vi "NISearchDLGKey.vi"(8 "error in":errorcluster, 10 "direction":i32, 11 "dlgH in":u64) -> (0 "error out":errorcluster, 3 "dlgH out":u64)   [LabVIEW 2023, in "GettingStartedWindow.lvlib"]
uses:
  <resource>/modes/FRC/GSW/GettingStartedWindow.lvlib
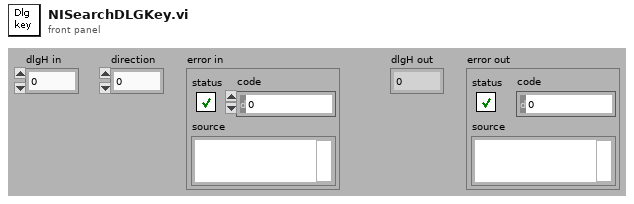
[diagram p1: front panel]
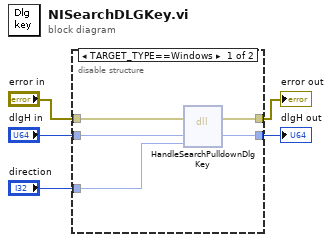
[diagram p0: block diagram]
diagram:
  n1 = disable-structure shown="TARGET_TYPE==Windows" {
    disable-tunnel: [w10 w11] -> w5
    disable-tunnel: [w9 w12] -> w4
    disable-tunnel: "dlgH in" -> [w8 w11]
    disable-tunnel: "error in" -> [w7 w12]
    disable-tunnel: "direction" -> [w6 _]
    frame condition #0 {
      n2 = dll-call lib="LabVIEW" fn="HandleSearchPulldownDlgKey"(error in=w7, "dlgH"=w8, "direction"=w6) -> (error out=w9:errorcluster, "dlgH"=w10:u64)  [unwired: 4 in, 1 out]
    }
    frame condition #1 (active) {
    }
  }
  "dlgH out" <- w5
  "error out" <- w4
